vi "libssh2_keepalive_send.vi"(8 "error in (no error)":errorcluster, 11 "session":T1) -> (0 "error out":errorcluster, 2 "seconds to next":i32)   [LabVIEW 2017, in "libssh2.lvlib"]
doc: "Send a keep-alive message if needed.\n\n<B>seconds to next</B> indicates how many seconds the caller can sleep before the next keep-alive message is due."
uses:
  libssh2.lvlib
  Session Refnum.ctl
  Not A Session.vi
  <vilib>/Utility/error.llb/Error Cluster From Error Code.vi
  Global Settings.vi
  Read Session Refnum.vi
  <vilib>/Utility/semaphor.llb/Acquire Semaphore.vi
  <vilib>/Utility/semaphor.llb/Release Semaphore.vi
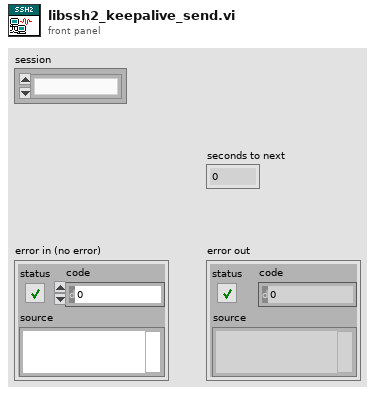
[diagram p1: front panel]
types:
  T1 = typedef "libssh2.lvlib/Session Refnum.ctl" = refnum<k1>
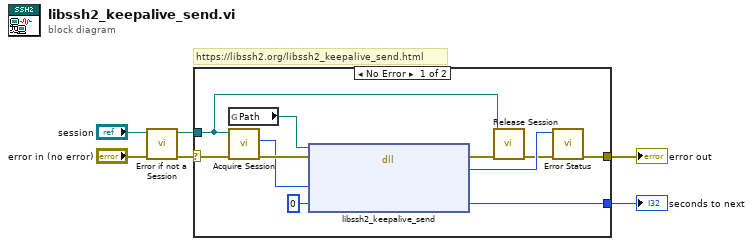
[diagram p0: block diagram]
diagram:
  # "https://libssh2.org/libssh2_keepalive_send.html"
  n1 = call "Error if not a Session.vi"("error in (no error)"="error in (no error)", "session"="session") -> ("error out"=w4:errorcluster, "session out"=w2:T1)  [unwired: 8 in]
  n2 = case shown="No Error" w4 {
    selector: w4 -> [w16 w18]
    tunnel: [w11 w18] -> w6
    tunnel: w2 -> [w7 _]
    tunnel: [w12 _] -> w1
    frame No Error {
      n3 = global read "Global Settings.vi" "Path"() -> (w13:path)
      n4 = call "Acquire Session.vi"("error in (no error)"=w16, "session"=w7) -> ("error out"=w15:errorcluster, "LIBSSH2_SESSION*"=w14:u64)  [unwired: 7 in, 1 out]
      n5 = dll-call lib="?" fn="libssh2_keepalive_send"(path in=w13, error in=w15, "session"=w14, "seconds_to_next"=0) -> (error out=w17:errorcluster, "return value"=w10:i32, "seconds_to_next"=w12:i32)  [unwired: 2 in, 1 out]
      n6 = call "Release Session.vi"("error in (no error)"=w17, "session"=w7) -> ("error out"=w8:errorcluster)  [unwired: 9 in]
      n7 = call "Error Status.vi"("error in (no error)"=w8, "return value"=w10) -> ("error out"=w11:errorcluster)  [unwired: 8 in, 1 out]
    }
    frame Error {
    }
  }
  "error out" <- w6
  "seconds to next" <- w1
